vi "Load.vi"(8 "error in (no error)":errorcluster, 11 "Tool in":refnum<class "MockTool.lvclass">) -> (0 "error out":errorcluster, 2 "OpenTool":variant, 3 "Tool out":refnum<class "MockTool.lvclass">)   [LabVIEW 2017, in "MockTool.lvclass"]
uses:
  MockTool.lvclass
  <vilib>/LVH/i3 JSON/i3-json.lvlib
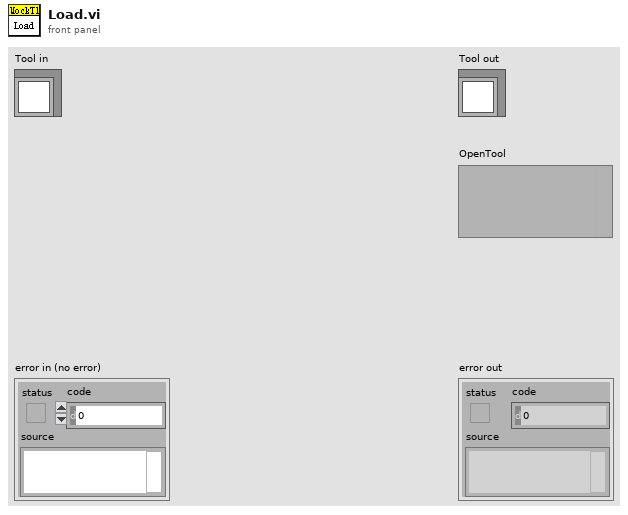
[diagram p1: front panel]
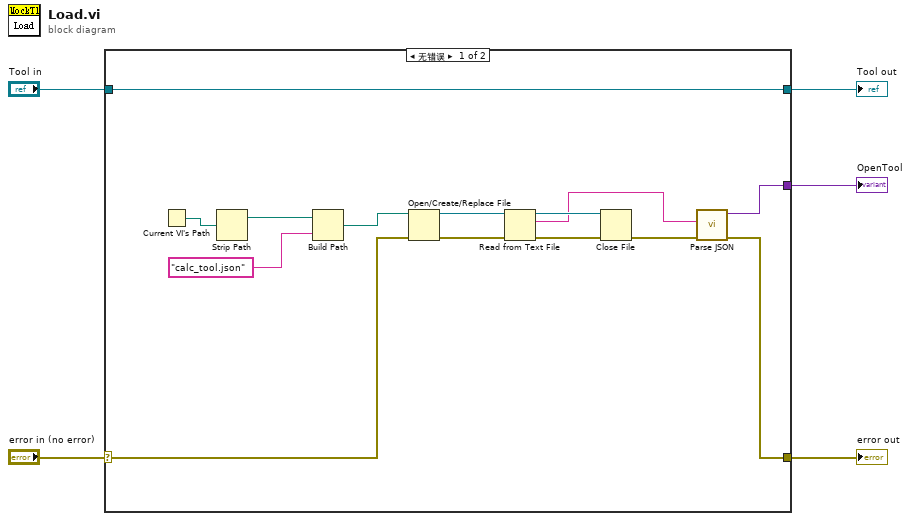
[diagram p0: block diagram]
diagram:
  n1 = case shown="无错误" "error in (no error)" {
    selector: "error in (no error)" -> [w11 w20]
    tunnel: [w13 _] -> w4
    tunnel: [w12 w21] -> w3
    tunnel: "Tool in" -> [w12 w21]
    tunnel: [w10 w20] -> w1
    frame No Error {
      n2 = Current VI's Path() -> (path=w9:path)
      n3 = Strip Path(path=w9) -> (stripped path=w7:path)  [unwired: 1 out]
      n4 = Build Path(base path=w7, name or relative path="calc_tool.json" ("名称或相对路径")) -> (appended path=w6:path)
      n5 = Open/Create/Replace File(file path (use dialog)=w6, error in=w11) -> (refnum out=w19:refnum<file>, error out=w18:errorcluster)  [unwired: 4 in, 1 out]
      n6 = Read from Text File(file (use dialog)=w19, error in=w18) -> (refnum out=w17:refnum<file>, text=w15:string, error out=w16:errorcluster)  [unwired: 2 in, 1 out]
      n7 = Close File(refnum=w17, error in=w16) -> (error out=w14:errorcluster)  [unwired: 1 out]
      n8 = call <vilib>:"Parse JSON.vi"("error in (no error)"=w14, "JSON String"=w15) -> ("error out"=w10:errorcluster, "JSON Tree"=w13:variant)  [unwired: 6 in, 2 out]
    }
    frame Error {
    }
  }
  "Tool out" <- w3
  "error out" <- w1
  "OpenTool" <- w4
